vi "VI control v4.0.vi"() -> ()   [LabVIEW 2021]
uses:
  <vilib>/DAQmx/read.llb/DAQmx Read (Counter DBL 1Chan 1Samp).vi
  <vilib>/DAQmx/write.llb/DAQmx Write (Analog DBL 1Chan 1Samp).vi
  <vilib>/DAQmx/write.llb/DAQmx Write (Digital 1D Bool 1Chan 1Samp).vi
  <vilib>/DAQmx/create/channels.llb/DAQmx Create Channel (CI-Position-Angular Encoder).vi
  <vilib>/DAQmx/create/channels.llb/DAQmx Create Channel (AO-Voltage-Basic).vi
  <vilib>/DAQmx/create/channels.llb/DAQmx Create Channel (DO-Digital Output).vi
  <vilib>/DAQmx/miscellaneous.llb/DAQmx Fill In Error Info.vi
  <vilib>/Utility/file.llb/Write Delimited Spreadsheet (DBL).vi
  <resource>/objmgr/daqmx.rc
panel:
  out "Energía":cluster{"E":dbl, "Eref":dbl}(graph)={"E"=1.000973101508098, "Eref"=1.02}
  in  "Path":path=path "C:/Users/labfisica/Documents/GitHub/Codigo_Proyecto_Pendulo/Logs/pruebas_vi_control_v4/p9.txt"
  out "Energia":dbl=1.000973101508098
  in  "Subir Péndulo":bool=TRUE
  in  "limcap":dbl
  in  "tauC":dbl=0.19
  in  "Tp":dbl=0.2
  in  "captura":dbl=8.0
  in  "ke":dbl=6.0
  in  "Eref":dbl=1.02
  in  "ref":dbl
  out "Error out":errorcluster
  in  "umin":dbl=0.02
  out "Velocidad angular [°/s]":dbl(graph)=10.744539511511496
  in  "AOmax":dbl=5.0
  in  "AO02":dbl=1.4
  in  "AO01":dbl=1.42
  in  "rT2":dbl=1.0
  in  "rT1":dbl=1.13
  in  "lines":tag="Dev1/port0/line2, Dev1/port0/line1"
  in  "counter":tag="Dev1/ctr0"
  in  "physical channels":tag="Dev1/ao0"
  out "AO [V]":dbl
  out "Estado":dbl=1.0
  out "Señal de Control u":cluster{"u":dbl, dbl}(graph)
  out "Ángulo [°]":cluster{"th":dbl, "ref":dbl, dbl, dbl}(graph)={"th"=-0.44999999999999996, "ref"=0.0, 2.0, -2.0}
  in  "Stop":bool
  in  "tauM":dbl=0.19
  in  "zeta":dbl=0.072
  in  "Th0":dbl=2.0
  in  "wn":dbl=4.185
  in  "Nv":dbl=-2346.0
  in  "Limite":dbl=1700.0
  in  "Kd":dbl=0.0085
  in  "Ventana":dbl=3.0
  in  "Ki":dbl=0.0143
  in  "Sentido":dbl=1.0
  in  "Kp":dbl=0.0159
  in  "Compensación":bool=TRUE
  in  "Simular":bool
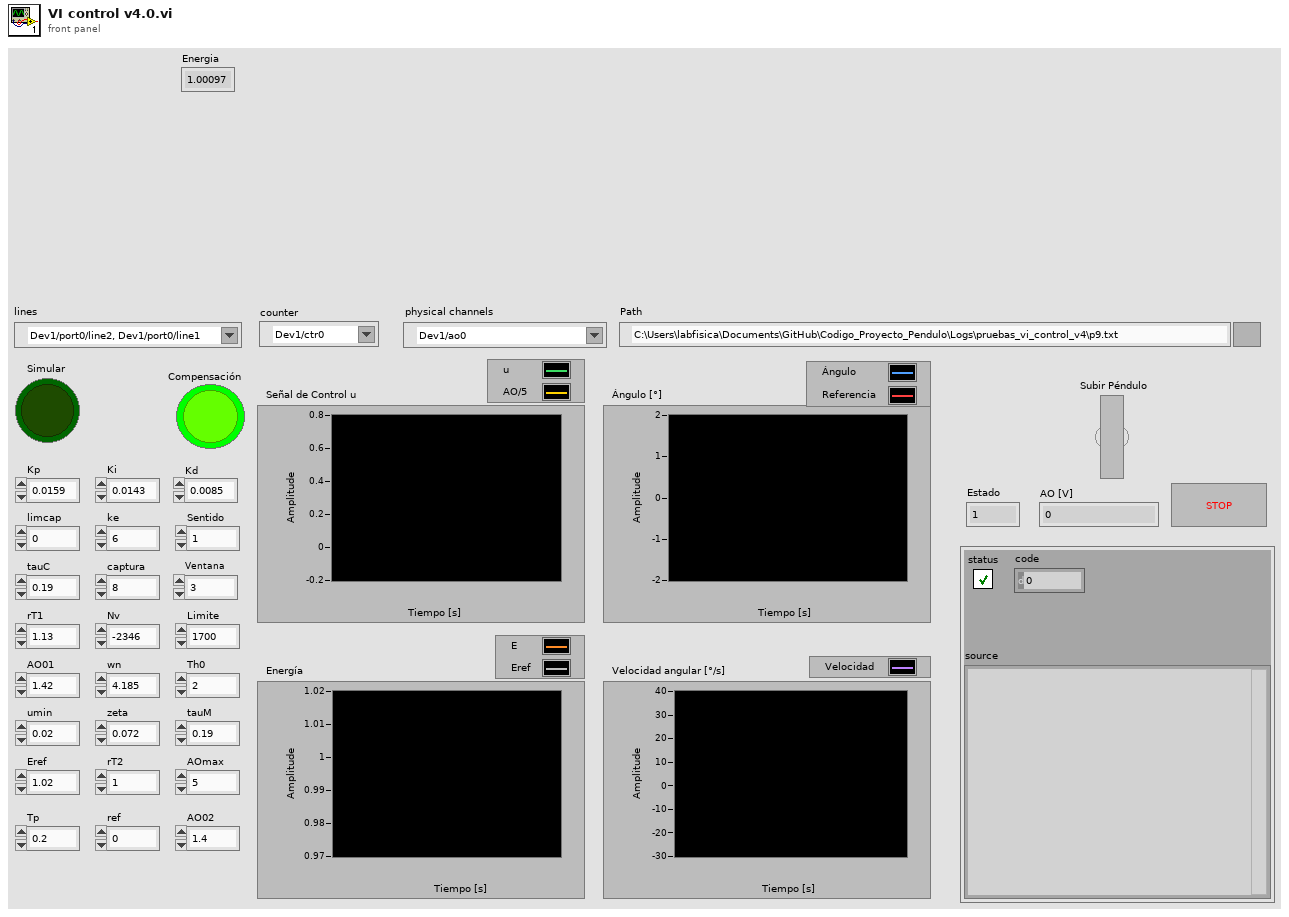
[diagram p1: front panel]
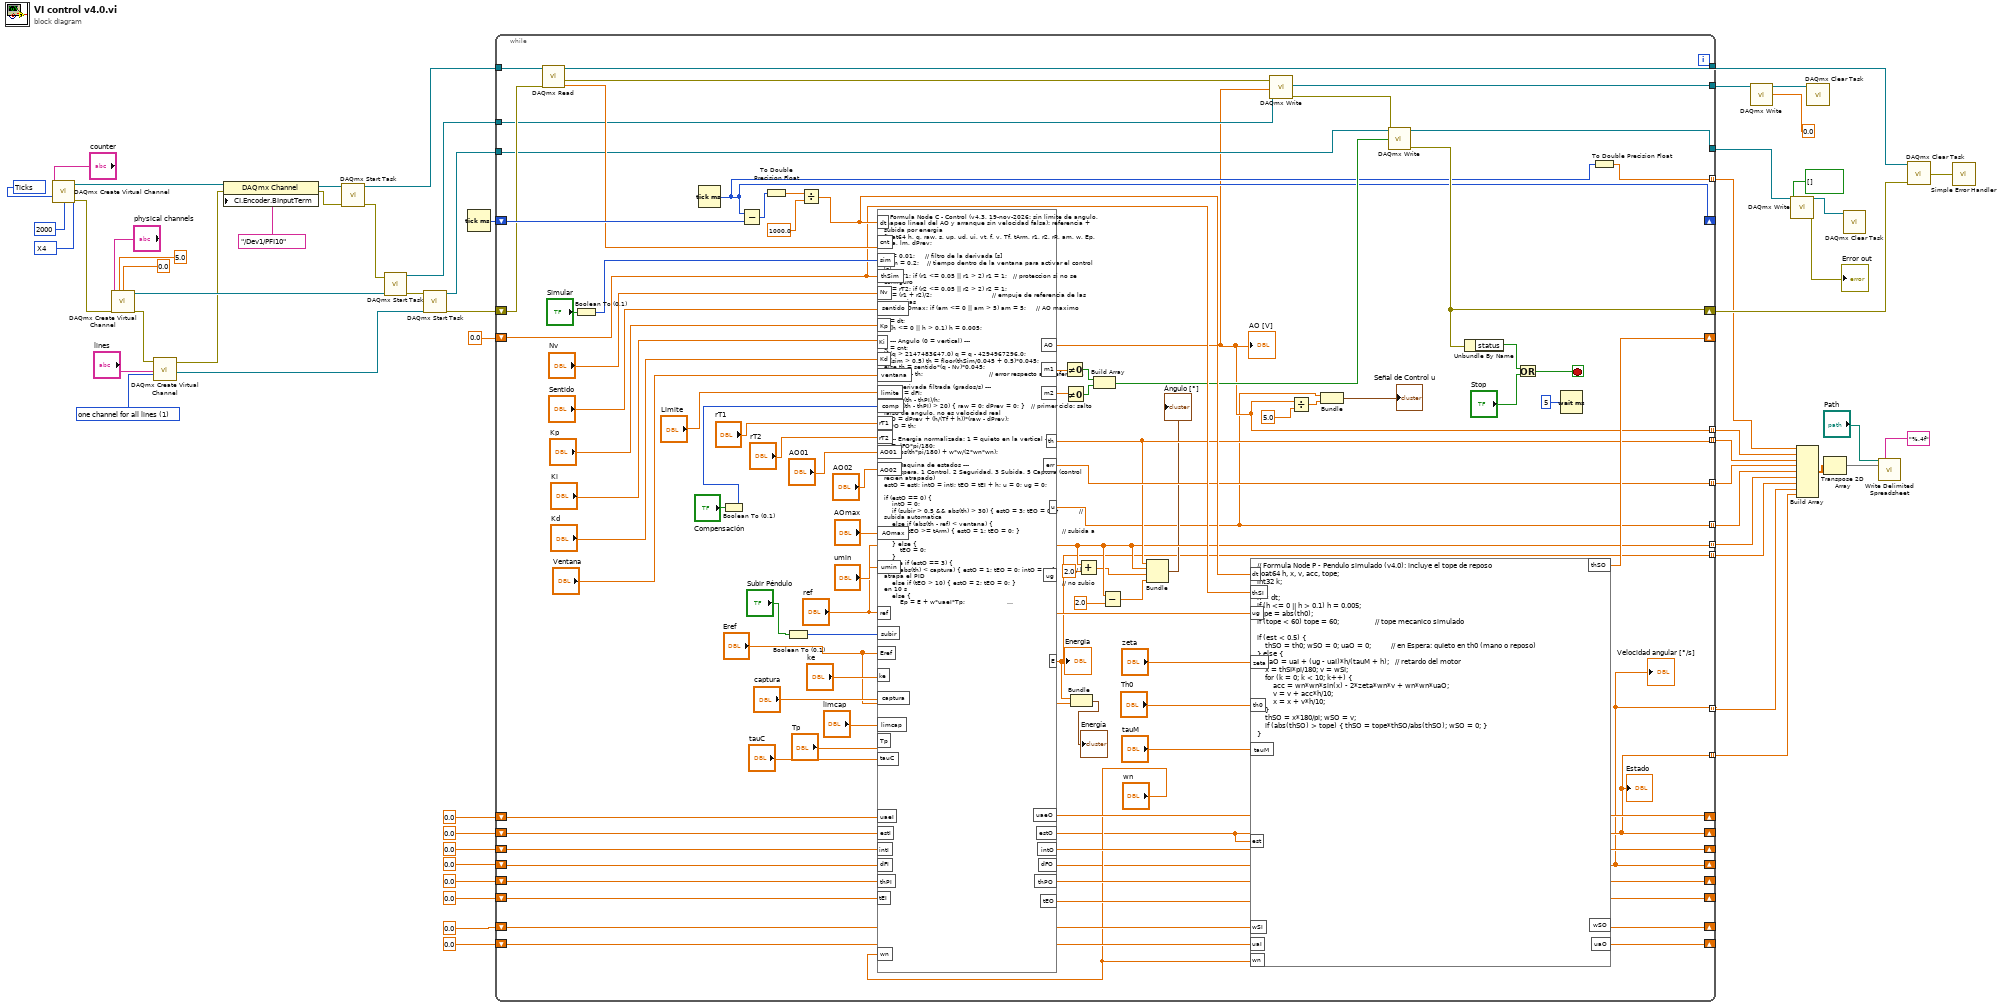
[diagram p0: block diagram]
diagram:
  w50 = 1 items=["one channel for each line", "one channel for all lines"] ("line grouping")
  w47 = 10304 items=["Degrees"=10146, "Radians"=10273, "Ticks"=10304, "From Custom Scale"=10065] ("units")
  w57 = 10092 items=["X1"=10090, "X2"=10091, "X4"=10092, "Two Pulse Counting"=10313] ("decoding type")
  n1 = call-poly <vilib>:"DAQmx Create Virtual Channel.vi"("counter"="counter", "decoding type"=w57, "units"=w47, "pulses per revolution"=u32 2000) -> ("task out"=w45:refnum<k21>, "error out"=w42:errorcluster)  [unwired: 10 in]
  n2 = call-poly <vilib>:"DAQmx Create Virtual Channel.vi"("maximum value"=5.0, "minimum value"=0.0, "physical channels"="physical channels", "error in"=w42) -> ("task out"=w49:refnum<k21>, "error out"=w41:errorcluster)  [unwired: 10 in]
  n3 = call-poly <vilib>:"DAQmx Create Virtual Channel.vi"("lines"="lines", "line grouping"=w50, "error in"=w41) -> ("task out"=w48:refnum<k21>, "error out"=w40:errorcluster)  [unwired: 11 in]
  n4 = property class="DAQmx Channel"(reference=w45, error in=w40, "CI.Encoder.BInputTerm"=tag "/Dev1/PFI10") -> (reference out=w44:refnum<k21>, error out=w43:errorcluster)
  n5 = call <vilib>:"DAQmx Start Task.vi"("task/channels in"=w44, "error in"=w43) -> ("task out"=w36:refnum<k21>, "error out"=w39:errorcluster)  [unwired: 12 in]
  n6 = call <vilib>:"DAQmx Start Task.vi"("task/channels in"=w49, "error in"=w39) -> ("task out"=w26:refnum<k21>, "error out"=w38:errorcluster)  [unwired: 12 in]
  n7 = call <vilib>:"DAQmx Start Task.vi"("task/channels in"=w48, "error in"=w38) -> ("task out"=w25:refnum<k21>, "error out"=w37:errorcluster)  [unwired: 12 in]
  n8 = Tick Count (ms)() -> (millisecond timer value=w35:u32)
  n9 = while {
    shift-right: [w74] -> _
    shift-left: w35 -> [w146]
    shift-right: [w111] -> _
    shift-left: 0.0 -> [w112]
    shift-right: [w108] -> _
    shift-left: 0.0 -> [w110]
    shift-right: [w107] -> _
    shift-left: 0.0 -> [w109]
    shift-right: [w120] -> _
    shift-left: 0.0 -> [w121]
    shift-right: [w76] -> _
    shift-left: 0.0 -> [w125]
    shift-right: [w119] -> _
    shift-left: 0.0 -> [w122]
    shift-right: [w118] -> _
    shift-left: 0.0 -> [w124]
    shift-right: [w75] -> _
    shift-left: 0.0 -> [w123]
    shift-right: [w79] -> w22
    shift-left: w37 -> [w141]
    tunnel: w36 -> [w147]
    tunnel: w26 -> [w80]
    tunnel: w25 -> [w78]
    tunnel: [w94] -> w15
    tunnel: [w93] -> w14
    tunnel: [w92] -> w18
    shift-right: [w83] -> _
    shift-left: 0.0 -> [w84]
    tunnel: [w70] -> w13 mode=indexing
    tunnel: [w77] -> w12 mode=indexing
    tunnel: [w62] -> w11 mode=indexing
    tunnel: ["ref"] -> w6 mode=indexing
    tunnel: [w76] -> w2 mode=indexing
    tunnel: [w65] -> w5 mode=indexing
    tunnel: [w75] -> w3 mode=indexing
    tunnel: [w60] -> w4 mode=indexing
    tunnel: [w73] -> w1 mode=indexing
    stop <- w97 stop-if-true
    n10 = call-poly <vilib>:"DAQmx Read.vi"("task/channels in"=w147, "error in"=w141) -> ("task out"=w94:refnum<k21>, "data"=w145:dbl, "error out"=w106:errorcluster)  [unwired: 11 in]
    n11 = Boolean To (0,1)(Boolean="Simular") -> (0, 1=w139:i16)
    n12 = Tick Count (ms)() -> (millisecond timer value=w74:u32)
    n13 = Boolean To (0,1)(Boolean="Compensación") -> (0, 1=w137:i16)
    n14 = Subtract(x=w74, y=w146) -> (x-y=w144:u32)
    n15 = To Double Precision Float(number=w144) -> (double precision float=w143:dbl)
    n16 = Boolean To (0,1)(Boolean="Subir Péndulo") -> (0, 1=w86:i16)
    n17 = Divide(x=w143, y=1000.0) -> (x/y=w116:dbl)
    n18 = formula code="// Formula Node C - Control (v4.3, 19-nov-2026: sin limite de angulo, mapeo lineal del AO y arranque sin velocidad falsa): referencia + subida por energia\nfloat64 h, q, raw, s, up, ud, ui, vt, f, v, Tf, tArm, r1, r2, rR, am, w, Ep, d, a, lm, dPrev;\n\nTf = 0.01;     // filtro de la derivada [s]\ntArm = 0.2;    // tiempo dentro de la ventana para activar el control [s]\nr1 = rT1; if (r1 <= 0.05 || r1 > 2) r1 = 1;   // proteccion si no se configuro\nr2 = rT2; if (r2 <= 0.05 || r2 > 2) r2 = 1;\nrR = (r1 + r2)/2;                              // empuje de referencia de las ganancias\nam = AOmax; if (am <= 0 || am > 5) am = 5;     // AO maximo\n\nh = dt;\nif (h <= 0 || h > 0.1) h = 0.005;\n\n// --- Angulo (0 = vertical) ---\nq = cnt;\nif (q > 2147483647.0) q = q - 4294967296.0;\nif (sim > 0.5) th = floor(thSim/0.045 + 0.5)*0.045;\nelse th = sentido*(q - Nv)*0.045;\nerr = ref - th;                                 // error respecto a la referencia\n\n// --- Derivada filtrada (grados/s) ---\ndPrev = dFI;\nraw = (th - thPI)/h;\nif (abs(th - thPI) > 20) { raw = 0; dPrev = 0; }   // primer ciclo: salto falso de angulo, no es velocidad real\ndFO = dPrev + (h/(Tf + h))*(raw - dPrev);\nthPO = th;\n\n// --- Energia normalizada: 1 = quieto en la vertical ---\nw = dFO*pi/180;\nE = cos(th*pi/180) + w*w/(2*wn*wn);\n\n// --- Maquina de estados ---\n// 0 Espera, 1 Control, 2 Seguridad, 3 Subida, 5 Captura (control recien atrapado)\nestO = estI; intO = intI; tEO = tEI + h; u = 0; ug = 0;\n\nif (estO == 0) {\n    intO = 0;\n    if (subir > 0.5 && abs(th) > 30) { estO = 3; tEO = 0; }          // subida automatica\n    else if (abs(th - ref) < ventana) {\n        if (tEO >= tArm) { estO = 1; tEO = 0; }                     // subida a mano\n    } else {\n        tEO = 0;\n    }\n} else if (estO == 3) {\n    if (abs(th) < captura) { estO = 1; tEO = 0; intO = 0; }         // lo atrapa el PID\n    else if (tEO > 10) { estO = 2; tEO = 0; }                       // no subio en 10 s\n    else {\n        Ep = E + w*uaeI*Tp;                       // energia predicha (dE/dt = w*empuje)\n        if (th > 0) d = -1; else d = 1;           // empujar hacia la vertical\n        a = ke*(Eref - Ep);                       // falta energia: empuja; sobra: frena\n        if (a > 1) a = 1;\n        if (a < -1) a = -1;\n        u = d*a;\n        if (u > 0) ug = u*r1; else ug = u*r2;\n    }\n} else if (estO == 2) {\n    intO = 0;\n    if (tEO > 1) { estO = 0; tEO = 0; }\n}\n\nif (estO == 1 || estO == 5) {                     // control PID, sin limite de angulo (v4.1)\n    estO = 1;\n        s = 0;\n        if (comp > 0.5) s = sin(th*pi/180);       // compensacion de gravedad\n        up = Kp*err;\n        ud = -Kd*dFO;\n        ui = intO + Ki*err*h;\n        vt = rR*(up + ui + ud) - s;\n        if (vt > 0) f = vt/r1; else f = vt/r2;\n        if (abs(f) < 1) intO = ui;               // anti-windup\n        v = rR*(up + intO + ud) - s;\n        if (v > 0) { u = v/r1; if (u > 1) u = 1; ug = u*r1; }\n        else       { u = v/r2; if (u < -1) u = -1; ug = u*r2; }\n}\n\n// --- Zona muerta de u: con u muy pequeno no se enciende ningun motor ---\nif (abs(u) < umin) { u = 0; ug = 0; }\n\n// --- Estimacion del empuje real (retardo del motor), para la prediccion de energia ---\nuaeO = uaeI + (ug - uaeI)*h/(tauC + h);\n\n// --- Salidas al actuador ---\nAO = 0; m1 = 0; m2 = 0;\nif (estO == 1 || estO == 3 || estO == 5) {\n    if (u > 0) { m1 = 1; AO = AO01 + (am - AO01)*u; }        // mapeo lineal (curvas del 19-nov)\n    if (u < 0) { m2 = 1; AO = AO02 + (am - AO02)*(-u); }\n}"("cnt"=w145, "dt"=w116, "sim"=w139, "thSim"=w112, "Nv"="Nv", "sentido"="Sentido", "Kp"="Kp", "Ki"="Ki", "Kd"="Kd", "ventana"="Ventana", "limite"="Limite", "comp"=w137, "rT1"="rT1", "rT2"="rT2", "AO01"="AO01", "AO02"="AO02", "estI"=w125, "intI"=w124, "dFI"=w123, "thPI"=w122, "tEI"=w121, "AOmax"="AOmax", "umin"="umin", "ref"="ref", "subir"=w86, "Eref"="Eref", "ke"="ke", "captura"="captura", "limcap"="limcap", "Tp"="Tp", "tauC"="tauC", "wn"="wn", "uaeI"=w84) -> ("th"=w70:dbl, "err"=w77:dbl, "u"=w62:dbl, "ug"=w117:dbl, "AO"=w65:dbl, "m1"=w105:dbl, "m2"=w104:dbl, "estO"=w76:dbl, "intO"=w118:dbl, "dFO"=w75:dbl, "thPO"=w119:dbl, "tEO"=w120:dbl, "E"=w60:dbl, "uaeO"=w83:dbl)
    "Estado" <- w76
    "AO [V]" <- w65
    "Velocidad angular [°/s]" <- w75
    "Energia" <- w60
    n19 = Not Equal To 0?(x=w105) -> (x != 0?=w103:bool)
    n20 = Not Equal To 0?(x=w104) -> (x != 0?=w102:bool)
    n21 = Bundle("E"=w60, "Eref"="Eref") -> (→"Energía":cluster{"E":dbl, "Eref":dbl})  [unwired: 1 in]
    n22 = Add(x="ref", y=2.0) -> (x+y=w68:dbl)
    n23 = Build Array(w103, w102) -> (w81:bool[])
    n24 = Subtract(x="ref", y=2.0) -> (x-y=w67:dbl)
    n25 = Bundle("th"=w70, "ref"="ref", w68, w67) -> (→"Ángulo [°]":cluster{"th":dbl, "ref":dbl, dbl, dbl})  [unwired: 1 in]
    n26 = formula code="// Formula Node P - Pendulo simulado (v4.0): incluye el tope de reposo\nfloat64 h, x, v, acc, tope;\nint32 k;\n\nh = dt;\nif (h <= 0 || h > 0.1) h = 0.005;\ntope = abs(th0);\nif (tope < 60) tope = 60;                  // tope mecanico simulado\n\nif (est < 0.5) {\n    thSO = th0; wSO = 0; uaO = 0;          // en Espera: quieto en th0 (mano o reposo)\n} else {\n    uaO = uaI + (ug - uaI)*h/(tauM + h);   // retardo del motor\n    x = thSI*pi/180; v = wSI;\n    for (k = 0; k < 10; k++) {\n        acc = wn*wn*sin(x) - 2*zeta*wn*v + wn*wn*uaO;\n        v = v + acc*h/10;\n        x = x + v*h/10;\n    }\n    thSO = x*180/pi; wSO = v;\n    if (abs(thSO) > tope) { thSO = tope*thSO/abs(thSO); wSO = 0; }\n}"("est"=w76, "dt"=w116, "wn"="wn", "zeta"="zeta", "th0"="Th0", "tauM"="tauM", "thSI"=w112, "wSI"=w110, "uaI"=w109, "ug"=w117) -> ("thSO"=w111:dbl, "wSO"=w108:dbl, "uaO"=w107:dbl)
    n27 = call-poly <vilib>:"DAQmx Write.vi"("task/channels in"=w80, "data"=w65, "error in"=w106) -> ("task out"=w93:refnum<k21>, "error out"=w101:errorcluster)  [unwired: 10 in, 1 out]
    n28 = Divide(x=w65, y=5.0) -> (x/y=w63:dbl)
    n29 = Bundle("u"=w62, w63) -> (→"Señal de Control u":cluster{"u":dbl, dbl})  [unwired: 1 in]
    n30 = call-poly <vilib>:"DAQmx Write.vi"("task/channels in"=w78, "data"=w81, "error in"=w101) -> ("task out"=w92:refnum<k21>, "error out"=w79:errorcluster)  [unwired: 10 in, 1 out]
    n31 = Unbundle By Name(w79) -> ("status"=w99:bool)
    n32 = Or(x=w99, y="Stop") -> (x .or. y?=w97:bool)
    n33 = Wait (ms)(milliseconds to wait=u32 5) -> ()  [unwired: 1 out]
    n34 = To Double Precision Float(number=w74) -> (double precision float=w73:dbl)
  }
  n35 = call-poly <vilib>:"DAQmx Write.vi"("task/channels in"=w14, "data"=0.0) -> ("task out"=w21:refnum<k21>)  [unwired: 11 in, 2 out]
  n36 = call-poly <vilib>:"DAQmx Write.vi"("task/channels in"=w18, "data"=bool[] []) -> ("task out"=w20:refnum<k21>, "error out"=→"Error out":errorcluster)  [unwired: 11 in, 1 out]
  n37 = Build Array(w1, w5, w13, w12, w11, w6, w4, w3, w2) -> (w10:dbl[][])
  n38 = call <vilib>:"DAQmx Clear Task.vi"("task in"=w21) -> ()  [unwired: 14 in, 1 out]
  n39 = Transpose 2D Array(2D array=w10) -> (transposed array=w9:dbl[][])
  n40 = call <vilib>:"DAQmx Clear Task.vi"("task in"=w20) -> ()  [unwired: 14 in, 1 out]
  n41 = call-poly <vilib>:"Write Delimited Spreadsheet.vi"("file path (dialog if empty)"="Path", "format (%.3f)"="%.4f", "2D data"=w9) -> ()  [unwired: 11 in, 2 out]
  n42 = call <vilib>:"DAQmx Clear Task.vi"("task in"=w15, "error in"=w22) -> ("error out"=w19:errorcluster)  [unwired: 13 in]
  n43 = call <vilib>:"Simple Error Handler.vi"("error in (no error)"=w19) -> ()  [unwired: 4 in, 5 out]
